vi "Run All Tests in Project.vi"() -> ()   [LabVIEW 2020]
panel:
  out "error out":errorcluster
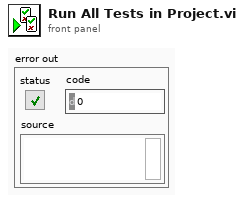
[diagram p1: front panel]
types:
  T1 = enum32{"Invalid", "Standard", "Closed", "Hidden", "Minimized", "Maximized"}
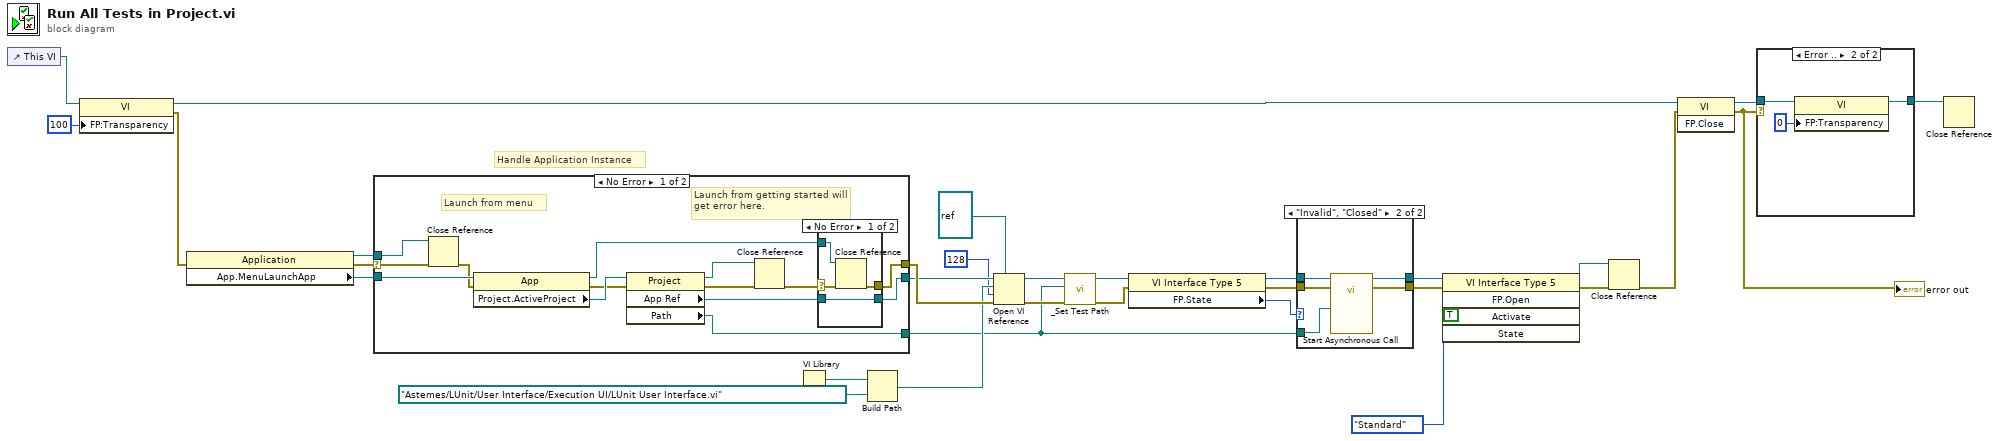
[diagram p0: block diagram]
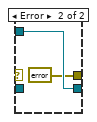
[diagram p2: hidden frame]
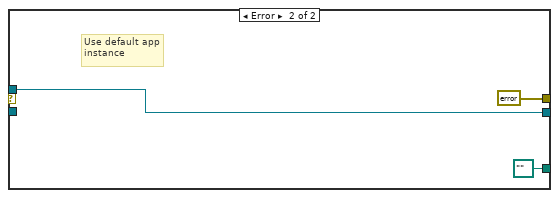
[diagram p3: hidden frame]
diagram:
  # "Handle Application Instance"
  n1 = control-ref of="This VI"() -> (w14:refnum<vi>)
  n2 = property class="VI"(reference=w14, "FP:Transparency"=u8 100 ("Front Panel Window:Transparency")) -> (reference out=w12:refnum<vi>, error out=w15:errorcluster)  [unwired: 1 in]
  n3 = property class="Application"(error in=w15) -> (reference out=w24:refnum<vi>, error out=w25:errorcluster, "App.MenuLaunchApp"=w26:refnum<vi>)  [unwired: 1 in]
  n4 = case shown="No Error" w25 {
    selector: w25 -> [w45 _]
    tunnel: [w38 w55] -> w28
    tunnel: w26 -> [w43 _]
    tunnel: w24 -> [w46 w55]
    tunnel: [w34 errorcluster {"status"=FALSE, "code"=0, "source"=""} ("error out")] -> w29
    tunnel: [w33 path "" ("Path")] -> w1
    frame No Error {
      # "Launch from getting started will get error here."
      # "Launch from menu"
      n5 = Close Reference(reference=w46, error in (no error)=w45) -> (error out=w42:errorcluster)
      n6 = property class="App"(reference=w43, error in=w42) -> (reference out=w41:refnum<vi>, error out=w39:errorcluster, "Project.ActiveProject"=w44:refnum<vi>)
      n7 = property class="Project"(reference=w44, error in=w39) -> (reference out=w40:refnum<vi>, error out=w36:errorcluster, "App Ref"=w37:refnum<vi>, "Path"=w33:path)
      n8 = Close Reference(reference=w40, error in (no error)=w36) -> (error out=w35:errorcluster)
      n9 = case shown="No Error" w35 {
        selector: w35 -> [w49 _]
        tunnel: w41 -> [w50 w52]
        tunnel: [w48 errorcluster {"status"=FALSE, "code"=0, "source"=""} ("error out")] -> w34
        tunnel: [w47 w52] -> w38
        tunnel: w37 -> [w47 _]
        frame No Error {
          n10 = Close Reference(reference=w50, error in (no error)=w49) -> (error out=w48:errorcluster)
        }
        frame Error {
        }
      }
    }
    frame Error {
      # "Use default app instance"
    }
  }
  n11 = VI Library() -> (path=w16:path)
  n12 = Build Path(base path=w16, name or relative path=path "Astemes/LUnit/User Interface/Execution UI/LUnit User Interface.vi") -> (appended path=w27:path)
  n13 = Open VI Reference(type specifier VI Refnum (for type only)=refnum<vi> refnum, application reference (local)=w28, vi path=w27, options=128, error in (no error)=w29) -> (vi reference=w5:refnum<vi>, error out=w2:errorcluster)  [unwired: 1 in]
  n14 = call "_Set Test Path.vi"("error in (no error)"=w2, "Path"=w1, "VI in"=w5) -> ("error out"=w3:errorcluster, "VI out"=w4:refnum<vi>)  [unwired: 7 in]
  n15 = property class="VI Interface Type 5"(reference=w4, error in=w3) -> (reference out=w20:refnum<vi>, error out=w19:errorcluster, "FP.State"=w18:T1)
  n16 = case shown="\"Invalid\", \"Closed\"" w18 {
    tunnel: w20 -> [w57 w62]
    tunnel: w19 -> [w56 w61]
    tunnel: [w57 w60] -> w7
    tunnel: [w56 w59] -> w6
    tunnel: w1 -> [_ w58]
    frame Default {
    }
    frame "Invalid", "Closed" {
      n17 = call-by-ref "Start Asynchronous Call"(reference=w62, error in=w61, "Test File Path"=w58) -> (reference out=w60:refnum<vi>, error out=w59:errorcluster)  [unwired: 11 in]
    }
  }
  n18 = invoke class="VI Interface Type 5" method="FP.Open"(reference=w7, error in=w6, "Activate"=TRUE ("Activate?"), "State"=T1."Standard") -> (reference out=w31:refnum<vi>, error out=w32:errorcluster)  [unwired: 1 in, 3 out]
  n19 = Close Reference(reference=w31, error in (no error)=w32) -> (error out=w10:errorcluster)
  n20 = invoke class="VI" method="FP.Close"(reference=w12, error in=w10) -> (reference out=w11:refnum<vi>, error out=w9:errorcluster)  [unwired: 1 in, 1 out]
  "error out" <- w9
  n21 = case shown="Error .." w9 {
    tunnel: [w63 w66] -> w30
    tunnel: w11 -> [w63 w65]
    frame No Error {
    }
    frame Error {
      n22 = property class="VI"(reference=w65, "FP:Transparency"=u8 0 ("Front Panel Window:Transparency")) -> (reference out=w66:refnum<vi>)  [unwired: 1 in, 1 out]
    }
  }
  n23 = Close Reference(reference=w30) -> ()  [unwired: 1 in, 1 out]
